vi "gdi32 DeleteDC.vi"(0 "hdc":u64, 11 "error in":errorcluster) -> (4 "return value":i32, 15 "error out":errorcluster)   [LabVIEW 2020, in "RemoteVI.lvlib"]
doc: "Deletes a device context created with gdi32 CreateCompatibleDC.vi, through gdi32.dll DeleteDC (stdcall, called in any thread). Do not use it on a DC from GetDC - release that with user32 ReleaseDC.vi. return value is non-zero on success. When error in carries an error the DLL is not called. Generated by scripts\\Build Win32 Wrappers.vi - do not edit by hand, rebuild it."
uses:
  RemoteVI.lvlib
  gdi32.dll
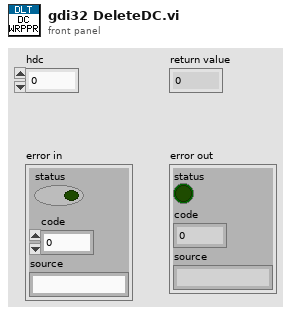
[diagram p1: front panel]
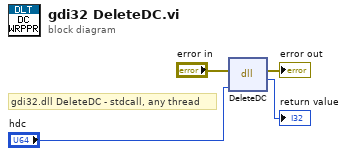
[diagram p0: block diagram]
diagram:
  # "gdi32.dll DeleteDC - stdcall, any thread"
  n1 = dll-call lib="gdi32.dll" fn="DeleteDC"(error in="error in", "hdc"="hdc") -> (error out=→"error out":errorcluster, →"return value":i32)  [unwired: 3 in, 1 out]
